vi "generate table.vi"(0 "TEC in":refnum<class "TEC configuration.lvclass">, 1 "from TEC":refnum<vi>, 2 "to TEC":refnum<vi>, 3 "avail tags":refnum<vi>, 5 "Pair in":refnum<class "TEC configuration.lvclass">, 7 "engine configuration in":refnum<class "engine configuration.lvclass">, 9 "paired engine in":refnum<class "engine configuration.lvclass">, 11 "error in":errorcluster, 12 "Filtering":string) -> (4 "TEC out":refnum<class "TEC configuration.lvclass">, 6 "pair out":refnum<class "TEC configuration.lvclass">, 8 "engine configuration out":refnum<class "engine configuration.lvclass">, 10 "paired engine out":refnum<class "engine configuration.lvclass">, 15 "error out":errorcluster)   [LabVIEW 2013, in "TEC editor node.lvclass"]
uses:
  TEC editor node.lvclass
  configuration/TEC configuration.lvclass
  <vilib>/NI/Module Execution Interface/Engine Configuration/engine configuration.lvclass
  <vilib>/NI/Tag Bus Module Framework/channel/channel classification.ctl
  <vilib>/NI/Tag Bus/tag/tag descriptor.lvclass/tag descriptor.ctl
  <vilib>/NI/Configuration Framework/serializable configuration/NISE_CEF_serializable configuration.lvclass/NISE_CEF_serializable configuration.ctl
  <vilib>/NI/Module Execution Interface/Engine Configuration/engine configuration.lvclass/engine configuration.ctl
  <vilib>/Utility/LVClass/Get LV Class Name.vi
  <vilib>/NI/Configuration Framework/error generator/NISE_error generator.vi
  <vilib>/NI/Tag Bus/tag/tag descriptor.lvclass
  <vilib>/NI/Tag Bus Module Framework/channel/TBM channel.lvclass
  <vilib>/NI/Configuration Framework/serializable configuration/NISE_CEF_serializable configuration.lvclass
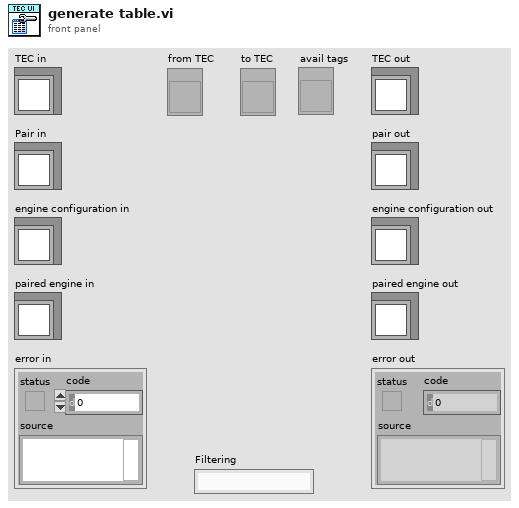
[diagram p1: front panel]
types:
  T1 = typedef "TBM channel.lvclass/channel classification.ctl" = enum16{"input data", "output data", "processing parameter", "processing result"}
  T2 = typedef "tag bus.lvlib/tag descriptor.lvclass/Data Type.ctl" = enum16{"Double", "Single", "I64", "I32", "I16", "I8", "U64", "U32", "U16", "U8", "Boolean", "String", "Array of Double", "Array of Single", "Array of I64", "Array of I32", "Array of I16", "Array of I8", "Array of U64", "Array of U32", "Array of U16", "Array of U8", "Array of Boolean", "Array of String"}
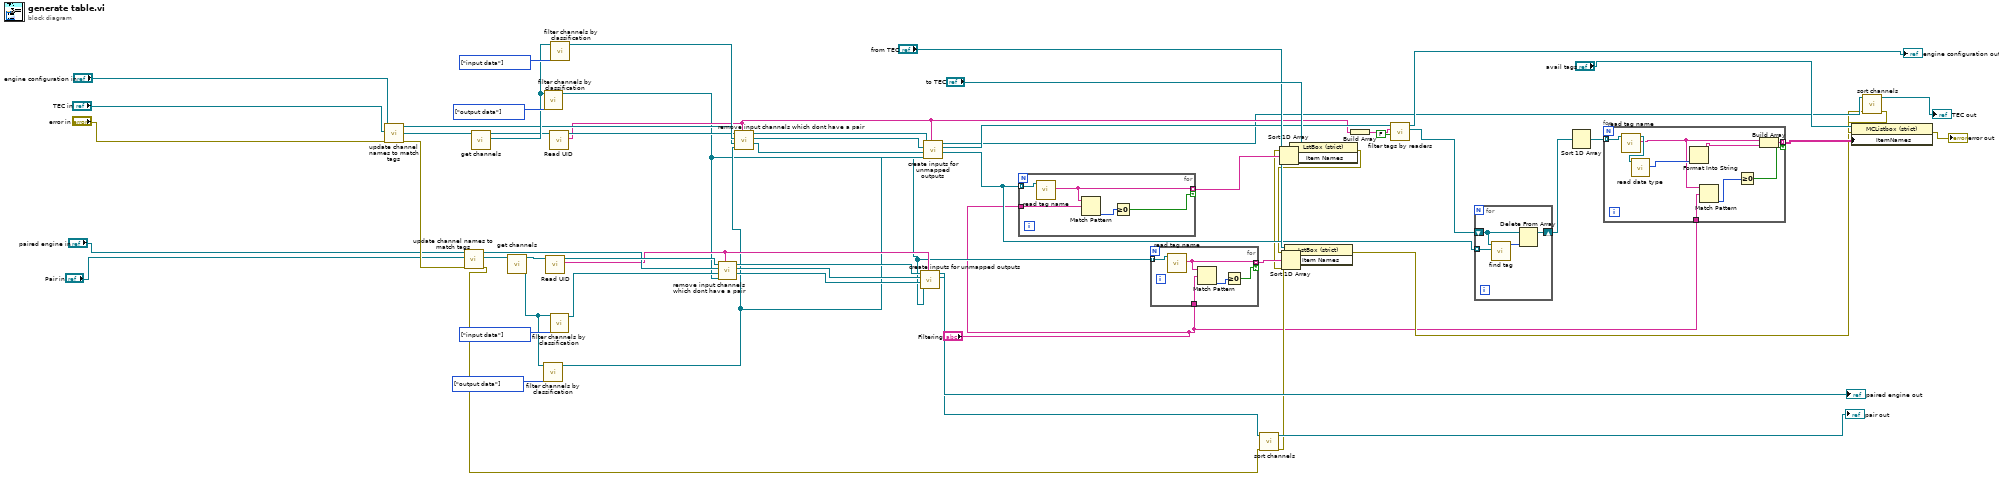
[diagram p0: block diagram]
diagram:
  w49 = T1[] [enum."output data"] items=["input data", "output data", "processing parameter", "processing result"] ("allowed classifications")
  w48 = T1[] [enum."input data"] items=["input data", "output data", "processing parameter", "processing result"] ("allowed classifications")
  w51 = T1[] [enum."output data"] items=["input data", "output data", "processing parameter", "processing result"] ("allowed classifications")
  w52 = T1[] [enum."input data"] items=["input data", "output data", "processing parameter", "processing result"] ("allowed classifications")
  n1 = call "update channel names to match tags.vi"("error in"="error in", "TEC in"="TEC in", "engine configuration in"="engine configuration in") -> ("error out"=w57:errorcluster, "TEC out"=w54:refnum<class "TEC configuration.lvclass">, "engine configuration out"=w46:refnum<class "engine configuration.lvclass">)  [unwired: 6 in]
  n2 = call "update channel names to match tags.vi"("error in"=w57, "TEC in"="Pair in", "engine configuration in"="paired engine in") -> ("error out"=w9:errorcluster, "TEC out"=w53:refnum<class "TEC configuration.lvclass">, "engine configuration out"=w39:refnum<class "engine configuration.lvclass">)  [unwired: 6 in]
  n3 = call-dynamic "get channels.vi"("TEC configuration in"=w54) -> ("channels"=w47:refnum<class "TBM channel.lvclass">[], "TEC configuration out"=w44:refnum<class "TEC configuration.lvclass">)  [unwired: 9 in]
  n4 = call-dynamic "get channels.vi"("TEC configuration in"=w53) -> ("channels"=w50:refnum<class "TBM channel.lvclass">[], "TEC configuration out"=w42:refnum<class "TEC configuration.lvclass">)  [unwired: 9 in]
  n5 = call <vilib>:"filter channels by classification.vi"("allowed classifications"=w51, "channels in"=w50) -> ("channels out"=w19:refnum<class "TBM channel.lvclass">[])  [unwired: 9 in]
  n6 = call <vilib>:"filter channels by classification.vi"("allowed classifications"=w49, "channels in"=w47) -> ("channels out"=w18:refnum<class "TBM channel.lvclass">[])  [unwired: 9 in]
  n7 = call <vilib>:"Read UID.vi"("configuration in"=w42) -> ("instance id"=w20:string, "configuration out"=w40:refnum<class "TEC configuration.lvclass">)  [unwired: 8 in, 1 out]
  n8 = call <vilib>:"Read UID.vi"("configuration in"=w44) -> ("instance id"=w21:string, "configuration out"=w43:refnum<class "TEC configuration.lvclass">)  [unwired: 8 in, 1 out]
  n9 = call <vilib>:"filter channels by classification.vi"("allowed classifications"=w52, "channels in"=w50) -> ("channels out"=w41:refnum<class "TBM channel.lvclass">[])  [unwired: 9 in]
  n10 = call <vilib>:"filter channels by classification.vi"("allowed classifications"=w48, "channels in"=w47) -> ("channels out"=w45:refnum<class "TBM channel.lvclass">[])  [unwired: 9 in]
  n11 = call "remove input channels which dont have a pair.vi"("instance id"=w20, "output channels"=w18, "input channels"=w41, "engine configuration in"=w39, "TEC configuration in"=w40) -> ("input channels out"=w33:refnum<class "TBM channel.lvclass">[], "engine configuration out"=w34:refnum<class "engine configuration.lvclass">, "TEC configuration out"=w35:refnum<class "TEC configuration.lvclass">)  [unwired: 4 in]
  n12 = call "remove input channels which dont have a pair.vi"("instance id"=w21, "output channels"=w19, "input channels"=w45, "engine configuration in"=w46, "TEC configuration in"=w43) -> ("input channels out"=w36:refnum<class "TBM channel.lvclass">[], "engine configuration out"=w37:refnum<class "engine configuration.lvclass">, "TEC configuration out"=w38:refnum<class "TEC configuration.lvclass">)  [unwired: 4 in]
  n13 = call "create inputs for unmapped outputs.vi"("module instance"=w20, "outputs"=w18, "input channels in"=w33, "engine configuration in"=w34, "TEC configuration in"=w35) -> ("engine configuration out"=→"paired engine out":refnum<class "engine configuration.lvclass">, "TEC configuration out"=w12:refnum<class "TEC configuration.lvclass">)  [unwired: 4 in, 1 out]
  n14 = call "create inputs for unmapped outputs.vi"("module instance"=w21, "outputs"=w19, "input channels in"=w36, "engine configuration in"=w37, "TEC configuration in"=w38) -> ("input channels out"=w15:refnum<class "TBM channel.lvclass">[], "engine configuration out"=w28:refnum<class "engine configuration.lvclass">, "TEC configuration out"=w14:refnum<class "TEC configuration.lvclass">)  [unwired: 4 in]
  n15 = for {
    tunnel: w15 -> [w65] mode=indexing
    tunnel: [w64] -> w31 mode=indexing if=w61
    tunnel: "Filtering" -> [w63]
    n16 = call <vilib>:"read tag name.vi"("system tag in"=w65) -> ("name"=w64:string)  [unwired: 8 in, 2 out]
    n17 = Match Pattern(string=w64, regular expression=w63) -> (offset past match=w62:i32)  [unwired: 1 in, 3 out]
    n18 = Greater Or Equal To 0?(x=w62) -> (x >= 0?=w61:bool)
  }
  n19 = for {
    tunnel: w18 -> [w70] mode=indexing
    tunnel: [w69] -> w30 mode=indexing if=w66
    tunnel: "Filtering" -> [w68]
    n20 = call <vilib>:"read tag name.vi"("system tag in"=w70) -> ("name"=w69:string)  [unwired: 8 in, 2 out]
    n21 = Match Pattern(string=w69, regular expression=w68) -> (offset past match=w67:i32)  [unwired: 1 in, 3 out]
    n22 = Greater Or Equal To 0?(x=w67) -> (x >= 0?=w66:bool)
  }
  n23 = call "sort channels.vi"("error in"=w9, "UDP Broadcaster Configuration in"=w12) -> ("error out"=w7:errorcluster, "UDP Broadcaster Configuration out"=→"pair out":refnum<class "TEC configuration.lvclass">)  [unwired: 8 in]
  n24 = Sort 1D Array(array=w31) -> (sorted array=w4:string[])
  n25 = Sort 1D Array(array=w30) -> (sorted array=w3:string[])
  n26 = property class="LstBox (strict)"(reference="to TEC", error in=w7, "Item Names"=w4) -> (error out=w6:errorcluster)  [unwired: 1 out]
  n27 = property class="LstBox (strict)"(reference="from TEC", error in=w6, "Item Names"=w3) -> (error out=w5:errorcluster)  [unwired: 1 out]
  n28 = Build Array(w21) -> (w27:string[])
  n29 = call <vilib>:"filter tags by readers.vi"("include? (default: exclude)"=FALSE, "reader modules"=w27, "engine configuration in"=w28) -> ("tag list"=w17:refnum<class "tag descriptor.lvclass">[], "engine configuration out"=→"engine configuration out":refnum<class "engine configuration.lvclass">)  [unwired: 7 in]
  n30 = for {
    shift-right: [w73] -> w16
    shift-left: w17 -> [w74]
    tunnel: w15 -> [w71] mode=indexing
    n31 = call <vilib>:"find tag.vi"("tag"=w71, "tags in"=w74) -> ("index"=w72:i32)  [unwired: 9 in]
    n32 = Delete From Array(array=w74, index=w72) -> (array with subset deleted=w73:refnum<class "tag descriptor.lvclass">[])  [unwired: 1 in, 1 out]
  }
  n33 = Sort 1D Array(array=w16) -> (sorted array=w2:refnum<class "tag descriptor.lvclass">[])
  n34 = for {
    tunnel: w2 -> [w83] mode=indexing
    tunnel: [w80] -> w25 mode=indexing if=w76
    tunnel: "Filtering" -> [w77]
    n35 = call <vilib>:"read tag name.vi"("system tag in"=w83) -> ("name"=w78:string, "system tag out"=w82:refnum<class "tag descriptor.lvclass">)  [unwired: 8 in, 1 out]
    n36 = call <vilib>:"read data type.vi"("system tag in"=w82) -> ("data type"=w81:T2)  [unwired: 8 in, 2 out]
    n37 = Format Into String(w81) -> (resulting string=w79:string)  [unwired: 3 in, 1 out]
    n38 = Match Pattern(string=w78, regular expression=w77) -> (offset past match=w75:i32)  [unwired: 1 in, 3 out]
    n39 = Greater Or Equal To 0?(x=w75) -> (x >= 0?=w76:bool)
    n40 = Build Array(w78, w79) -> (w80:string[])
  }
  n41 = call "sort channels.vi"("error in"=w5, "UDP Broadcaster Configuration in"=w14) -> ("error out"=w10:errorcluster, "UDP Broadcaster Configuration out"=→"TEC out":refnum<class "TEC configuration.lvclass">)  [unwired: 8 in]
  n42 = property class="MCListbox (strict)"(reference="avail tags", error in=w10, "ItemNames"=w25) -> (error out=→"error out":errorcluster)  [unwired: 1 out]
